vi "Highligth Selected Row.vi"(8 "error in":errorcluster, 9 "Current Row":i32, 11 "Table in":refnum<vi>) -> (0 "error out":errorcluster)   [LabVIEW 2025, in "Automotive Ethernet Bus Monitor UI.lvlib"]
doc: "Set currently selected row as the highlighted one, and remove the highligth from the previous one."
uses:
  Automotive Ethernet Bus Monitor UI.lvlib
  <vilib>/Utility/miscctls.llb/LVRowAndColumnTypeDef.ctl
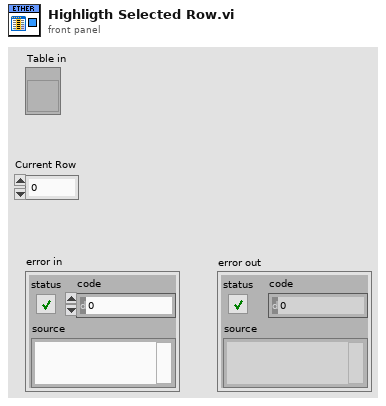
[diagram p1: front panel]
types:
  T1 = typedef "LVRowAndColumnTypeDef.ctl" = cluster{"Row":i32, "Column":i32}
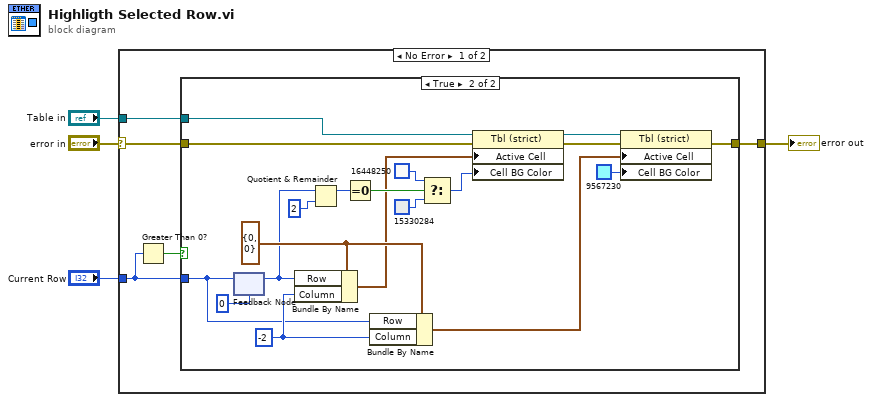
[diagram p0: block diagram]
diagram:
  n1 = case shown="No Error" "error in" {
    selector: "error in" -> [w7 w30]
    tunnel: [w9 w30] -> w4
    tunnel: "Table in" -> [w8 _]
    tunnel: "Current Row" -> [w6 _]
    frame No Error {
      n2 = Greater Than 0?(x=w6) -> (x > 0?=w5:bool)
      n3 = case shown="True" w5 {
        tunnel: [w10 w29] -> w9
        tunnel: w8 -> [_ w26]
        tunnel: w7 -> [w10 w21]
        tunnel: w6 -> [_ w19]
        frame False {
        }
        frame True {
          w25 = -2 ("Column")
          w20 = T1 {"Row"=0, "Column"=0} ("Active Cell:Active Cell")
          n4 = feedback #1(0 ("Row")) -> (w14:i32)
          n5 = feedback-in #1(w19) -> ()
          n6 = Bundle By Name(cluster=w20, "Row"=w14, "Column"=w25) -> (w11:T1)
          n7 = Quotient & Remainder(x=w14, y=2) -> (x-y*floor(x/y)=w17:i32)  [unwired: 1 out]
          n8 = Equal To 0?(x=w17) -> (x = 0?=w16:bool)
          n9 = Bundle By Name(cluster=w20, "Row"=w19, "Column"=w25) -> (w23:T1)
          n10 = Select(t=u32 16448250 ("Active Cell:Cell Background Color"), s=w16, f=u32 15330284 ("Alternate Row Background Color")) -> (s? t:f=w15:u32)
          n11 = property class="Tbl (strict)"(reference=w26, error in=w21, "Active Cell"=w11, "Cell BG Color"=w15) -> (reference out=w27:refnum<vi>, error out=w28:errorcluster)
          n12 = property class="Tbl (strict)"(reference=w27, error in=w28, "Active Cell"=w23, "Cell BG Color"=u32 9567230 ("Active Cell:Cell Background Color")) -> (error out=w29:errorcluster)  [unwired: 1 out]
        }
      }
    }
    frame Error {
    }
  }
  "error out" <- w4
